vi "Stop Log.vi"(7 "VolatusAPI in":refnum<class "VolatusAPI.lvclass">, 8 "error in (no error)":errorcluster, 9 "Target (All)":string, 10 "Log Group (All)":T1, 11 "GroupLoggingControl in":refnum<class "GroupLoggingControl.lvclass">) -> (0 "error out":errorcluster, 3 "GroupLoggingControl out":refnum<class "GroupLoggingControl.lvclass">)   [LabVIEW 2020, in "VolatusGUIElements.lvlib" / "GroupLoggingControl.lvclass"]
uses:
  GroupLoggingControl.lvclass
  Log Group.ctl
  Log Group Status.ctl
  Command Info.ctl
  Volatus/VolatusAPI/VolatusAPI.lvclass
  messages/StopLog/Data.ctl
  GroupLoggingControl.lvclass/GroupLoggingControl.ctl
  messages/StopLog/Class/Msg.lvclass/Msg.ctl
  Volatus/VolatusAPI/VolatusAPI.lvclass/VolatusAPI.ctl
  messages/StopLog/Class/Msg.lvclass
  C:/dev/lv20CE/relink/lv-protoc/LV-Proto/Message/Message.lvclass
  lv-vecto/Vecto/TCPMessageService/Send Message.vi
  <vilib>/Utility/error.llb/Error Cluster From Error Code.vi
  lv-protoc/LV-Proto/Message/Message.lvclass
  messages/StopLog/StopLog.lvlib
  C:/dev/lv20CE/relink/lv-volatus/messages/StopLog/Class/Msg.lvclass
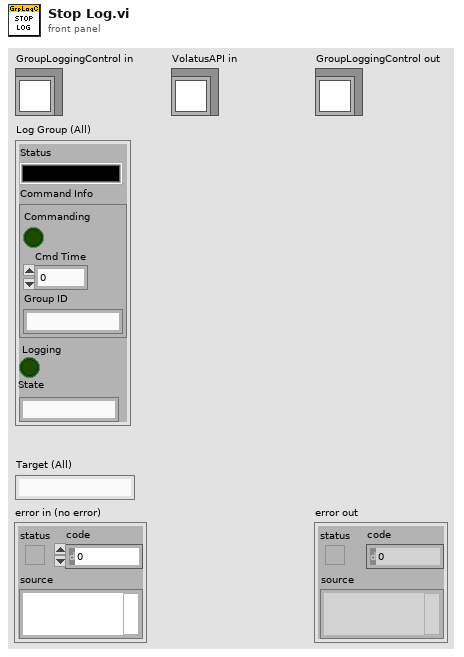
[diagram p1: front panel]
types:
  T1 = typedef "VolatusGUIElements.lvlib/GroupLoggingControl.lvclass/Log Group.ctl" = cluster{"Status":T2, "Command Info":T3, "Logging":bool, "State":string}
  T2 = typedef "VolatusGUIElements.lvlib/GroupLoggingControl.lvclass/Log Group Status.ctl" = cluster{"Group":string, "Group Color":u32, "Button":bool}
  T3 = typedef "VolatusGUIElements.lvlib/GroupLoggingControl.lvclass/Command Info.ctl" = cluster{"Commanding":bool, "Cmd Time":dbl, "Group ID":string}
  T4 = typedef "StopLog.lvlib/Data.ctl" = cluster{"reason":string, "groups":string[]}
  T5 = typedef "VolatusGUIElements.lvlib/GroupLoggingControl.lvclass/Status.ctl" = cluster{"Groups":T1[], "Targets":T6[]}
  T6 = typedef "VolatusGUIElements.lvlib/GroupLoggingControl.lvclass/Target Info.ctl" = cluster{"Node":string, "Node Color":u32, "Groups":T1[]}
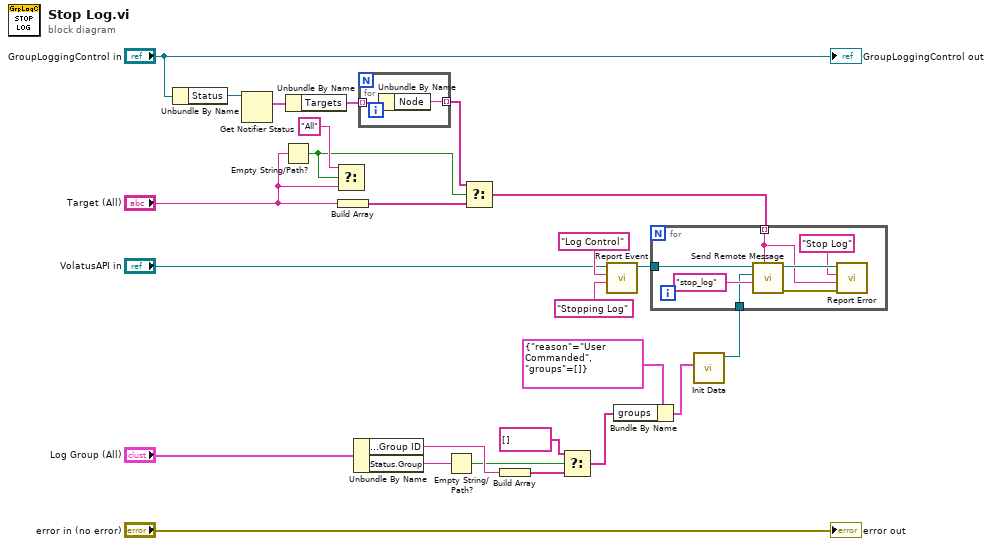
[diagram p0: block diagram]
diagram:
  n1 = Unbundle By Name("GroupLoggingControl in") -> ("Status"=w2:refnum<notifier>)
  n2 = Get Notifier Status(notifier=w2) -> (current notification=w1:T5)  [unwired: 1 in, 4 out]
  n3 = Empty String/Path?(string/path="Target (All)") -> (empty?=w17:bool)
  n4 = Unbundle By Name(w1) -> ("Targets"=w18:T6[])
  n5 = Select(t="All", s=w17, f="Target (All)") -> ()  [unwired: 1 out]
  n6 = Build Array("Target (All)") -> (w15:string[])
  n7 = Unbundle By Name("Log Group (All)") -> ("Command Info.Group ID"=w5:string, "Status.Group"=w10:string)
  n8 = for {
    tunnel: w18 -> [w27] mode=indexing
    tunnel: [w26] -> w16 mode=indexing
    n9 = Unbundle By Name(w27) -> ("Node"=w26:string)
  }
  n10 = Empty String/Path?(string/path=w10) -> (empty?=w4:bool)
  n11 = Select(t=w16, s=w17, f=w15) -> (s? t:f=w13:string[])
  n12 = Build Array(w5) -> (w9:string[])
  n13 = Select(t=string[] [], s=w4, f=w9) -> (s? t:f=w6:string[])
  n14 = call "Report Event.vi"("Message"="Stopping Log" ("Context"), "Context"="Log Control", "VolatusAPI in"="VolatusAPI in") -> ("VolatusAPI out"=w23:refnum<class "VolatusAPI.lvclass">)  [unwired: 7 in, 1 out]
  n15 = Bundle By Name(cluster=T4 {"reason"="User Commanded", "groups"=[]} ("Data"), "groups"=w6) -> (w11:T4)
  n16 = call "Init Data.vi"("Data"=w11) -> ("Msg out"=w24:refnum<class "Msg.lvclass">)  [unwired: 10 in]
  n17 = for {
    tunnel: w23 -> [w34]
    tunnel: w13 -> [w29] mode=indexing
    tunnel: w24 -> [w28]
    n18 = call "Send Remote Message.vi"("Target Name"=w29, "Message Type"="stop_log", "Message"=w28, "VolatusAPI in"=w34) -> ("error out"=w30:errorcluster, "VolatusAPI out"=w33:refnum<class "VolatusAPI.lvclass">)  [unwired: 6 in]
    n19 = call "Report Error.vi"("error in (no error)"=w30, "Message"=w29, "Context"="Stop Log", "VolatusAPI in"=w33) -> ()  [unwired: 6 in, 2 out]
  }
  "error out" <- "error in (no error)"
  "GroupLoggingControl out" <- "GroupLoggingControl in"
